vi "RDC-permittivity-handle_matrix.vi"(7 "basic data(open, short, water, ...)":T1[](array[typedef]), 11 "Data Array":T1[](array[typedef])) -> (3 "Common Format out":T1[](array[typedef]))   [LabVIEW 2020, in "RDC-Reflection_Data_Computation.lvlib"]
doc: "Splits Data Array into groups and runs RDC-permittivity-handle_all on each with its basic data. Returns all results."
uses:
  RDC-Reflection_Data_Computation.lvlib
  Reflector/RFH-common_data_format.ctl
  RDC-perm_calc_type.ctl
  Reflector/RFH-Reflection_File_Handler.lvlib
panel:
  out "32bit integer":i32
  out "x-y*floor(x/y)":i32
  out "floor(x/y)":i32
  out "x = 0?":bool
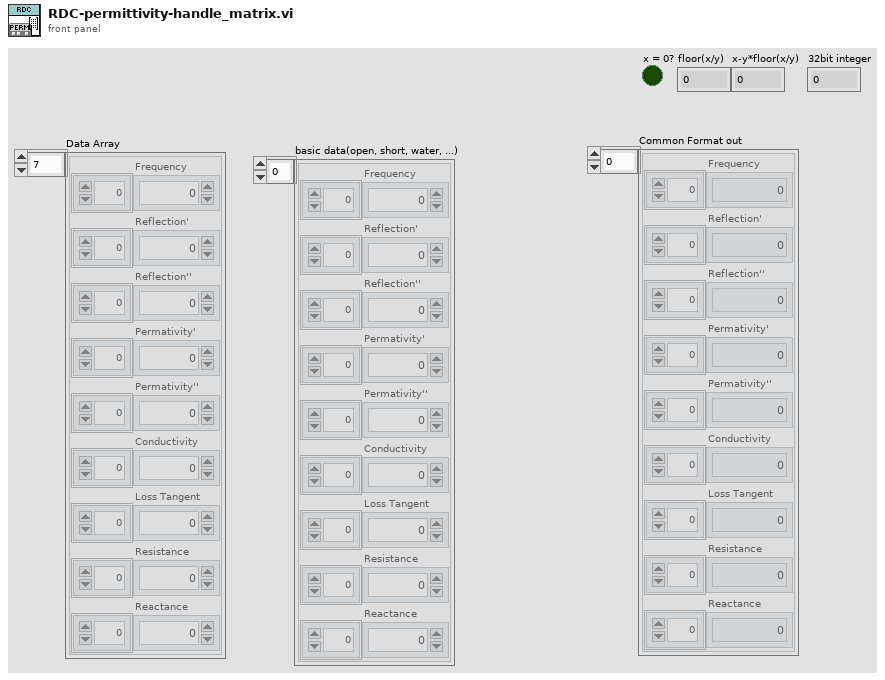
[diagram p1: front panel]
types:
  T1 = typedef "RFH-Reflection_File_Handler.lvlib/RFH-common_data_format.ctl" = cluster{"Frequency":dbl[], "Reflection'":dbl[], "Reflection''":dbl[], "Permativity'":dbl[], "Permativity''":dbl[], "Conductivity":dbl[], "Loss Tangent":dbl[], "Resistance":dbl[], "Reactance":dbl[]}
  T2 = typedef "RDC-Reflection_Data_Computation.lvlib/RDC-perm_calc_type.ctl" = enum16{"Basic", "Capacative", "Advance", "Bilinear", "Size"}
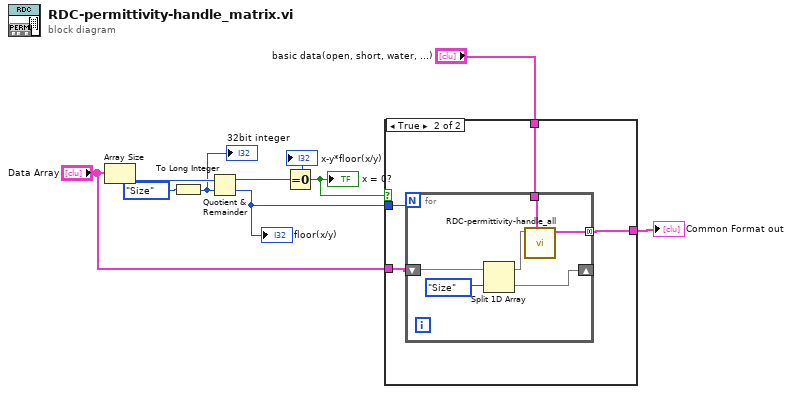
[diagram p0: block diagram]
diagram:
  n1 = Array Size(array="Data Array") -> (size(s)=w9:i32)
  n2 = To Long Integer(number=RDC-perm_calc_type."Size" ("Perm calc type")) -> (32bit integer=w7:i32)
  "32bit integer" <- w7
  n3 = Quotient & Remainder(x=w9, y=w7) -> (x-y*floor(x/y)=w6:i32, floor(x/y)=w5:i32)
  "floor(x/y)" <- w5
  "x-y*floor(x/y)" <- w6
  n4 = Equal To 0?(x=w6) -> (x = 0?=w2:bool)
  "x = 0?" <- w2
  n5 = case shown="True" w2 {
    tunnel: w5 -> [_ w14]
    tunnel: "Data Array" -> [w10 w13]
    tunnel: "basic data(open, short, water, ...)" -> [_ w12]
    tunnel: [w10 w11] -> w1
    frame False {
    }
    frame True {
      n6 = for {
        N: w14 -> [_]
        shift-right: [w18] -> _
        shift-left: w13 -> [w19]
        tunnel: w12 -> [w15]
        tunnel: [w16] -> w11 mode=concatenating
        n7 = Split 1D Array(array=w19, index=RDC-perm_calc_type."Size" ("Perm calc type")) -> (first subarray=w17:T1[], second subarray=w18:T1[])
        n8 = call "RDC-permittivity-handle_all.vi"("basic data(open, short, water, ...)"=w15, "Data Array"=w17) -> ("Common Format out"=w16:T1[])  [unwired: 9 in]
      }
    }
  }
  "Common Format out" <- w1
